vi "ZM-HWM-init.vi"(8 "error in":errorcluster, 11 "ZM-HWM-hardware_manager in":refnum<class "ZM-HWM-hardware_manager.lvclass">) -> (0 "error out":errorcluster, 2 "Event Registration Refnum":refnum<event-registration>, 3 "ZM-HWM-hardware_manager out":refnum<class "ZM-HWM-hardware_manager.lvclass">)   [LabVIEW 2020, in "ZM-HWM-hardware_manager.lvlib" / "ZM-HWM-hardware_manager.lvclass"]
doc: "Init of the hardware manager, run in Actor Core before Call Parent: registers for the stop user event and hands the registration to ZM-HWM-helperAcquisition. Registering before the actor runs means a stop is never lost. An incoming or registration error goes on into Call Parent, so the actor stops at once."
uses:
  ZM-HWM-hardware_manager.lvclass
  ZM-HWM-hardware_manager.lvclass/ZM-HWM-hardware_manager.ctl
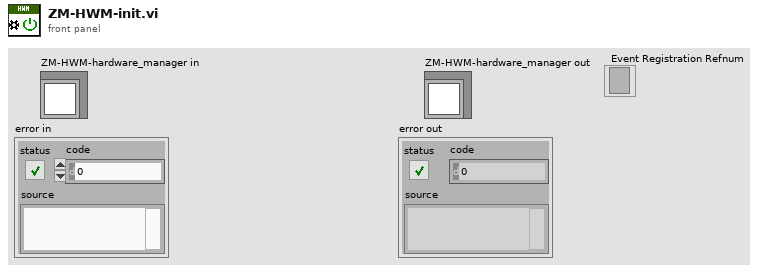
[diagram p1: front panel]
types:
  T1 = typedef "ZM-HWM-hardware_manager.lvlib/ZM-HWM-hardware_manager.lvclass/ZM-HWM-EVENTS.ctl" = cluster{"stop":refnum<user-event>}
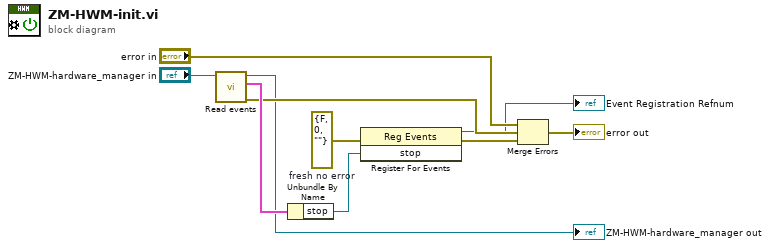
[diagram p0: block diagram]
diagram:
  w8 = errorcluster {"status"=FALSE, "code"=0, "source"=""}  # fresh no error
  n1 = call "Read events.vi"("ZM-HWM-hardware_manager in"="ZM-HWM-hardware_manager in") -> ("error out"=w5:errorcluster, "ZM-HWM-EVENTS"=w9:T1, "ZM-HWM-hardware_manager out"=→"ZM-HWM-hardware_manager out":refnum<class "ZM-HWM-hardware_manager.lvclass">)  [unwired: 8 in]
  n2 = Unbundle By Name(w9) -> ("stop"=w7:refnum<user-event>)
  n3 = register-events(error in=w8, w7) -> (reference out=→"Event Registration Refnum":refnum<event-registration>, error out=w4:errorcluster)  [unwired: 1 in]
  n4 = Merge Errors("error in", w5, w4) -> (→"error out":errorcluster)
